vi "Set User Data Folder Internal.vi"(8 "error in (no error)":errorcluster, 10 "User Data":path, 11 "Webview2":refnum<k24>) -> (0 "error out":errorcluster, 3 "Webview2":refnum<k24>)   [LabVIEW 2020, in "WebView2.lvlib" / "WebView2 Control.lvclass"]
uses:
  WebView2 Control.lvclass
  C:/Users/Simon/Documents/GitHub/LV-WebView2/Source/Libs/Microsoft.Web.WebView2.WinForms.dll
  Libs/Microsoft.Web.WebView2.WinForms.dll
  WebView2 Control.lvclass/WebView2 Control.ctl
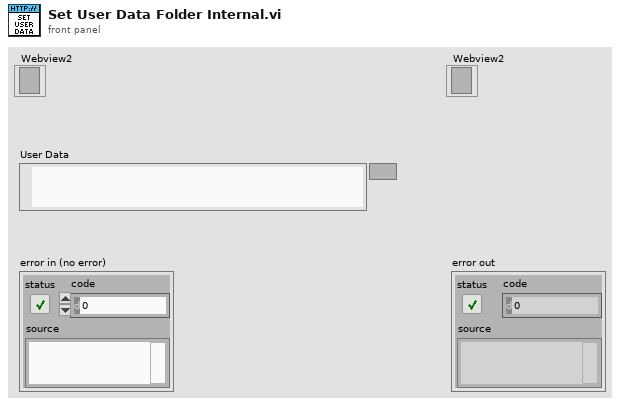
[diagram p1: front panel]
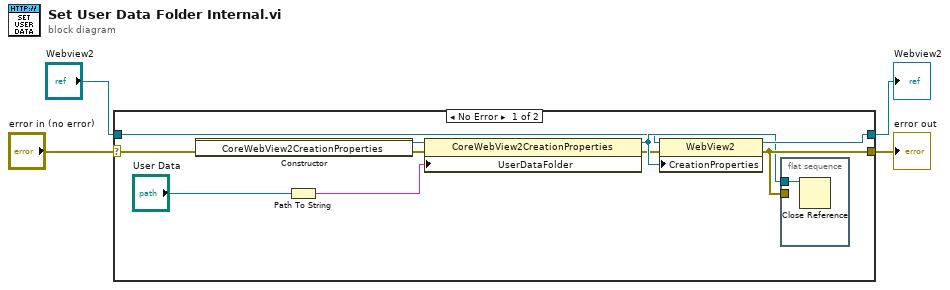
[diagram p0: block diagram]
diagram:
  n1 = case shown="No Error" "error in (no error)" {
    selector: "error in (no error)" -> [w10 w17]
    tunnel: [w14 w16] -> w4
    tunnel: "Webview2" -> [w9 w16]
    tunnel: [w13 w17] -> w1
    frame No Error {
      n2 = constructor class="CoreWebView2CreationProperties"(error in=w10) -> (reference out=w7:refnum<k24>, error out=w6:errorcluster)  [unwired: 2 in, 1 out]
      n3 = Path To String(path="User Data") -> (string=w5:string)
      n4 = property class="CoreWebView2CreationProperties"(reference=w7, error in=w6, "UserDataFolder"=w5) -> (reference out=w12:refnum<k24>, error out=w8:errorcluster)
      n5 = property class="WebView2"(reference=w9, error in=w8, "CreationProperties"=w12) -> (reference out=w14:refnum<k24>, error out=w13:errorcluster)
      n6 = flat-sequence {
        tunnel: w13 -> [_]
        tunnel: w12 -> [w15]
        frame #0 {
          n7 = Close Reference(reference=w15) -> ()  [unwired: 1 in, 1 out]
        }
      }
    }
    frame Error {
    }
  }
  "error out" <- w1
  "Webview2" <- w4
